vi "test3-FirstChainNodeProcessesAllowedMessages.vi"(8 "error in (no error)":errorcluster, 11 "TestCase in":refnum<class "testcase-CSMChainMode.lvclass">) -> (0 "error out":errorcluster, 3 "TestCase out":refnum<class "testcase-CSMChainMode.lvclass">)   [LabVIEW 2017, in "testcase-CSMChainMode.lvclass"]
uses:
  testcase-CSMChainMode.lvclass
  <vilib>/addons/_JKI Toolkits/VI Tester/TestCase.llb/TestCase.lvclass
  src/user.lib/_NEVSTOP/Communicable State Machine(CSM)/Communicable State Machine.lvlib
  C:/Program Files (x86)/National Instruments/LabVIEW 2017/vi.lib/addons/_JKI Toolkits/VI Tester/TestCase.llb/TestCase.lvclass
panel:
  out "LoopCount":i32
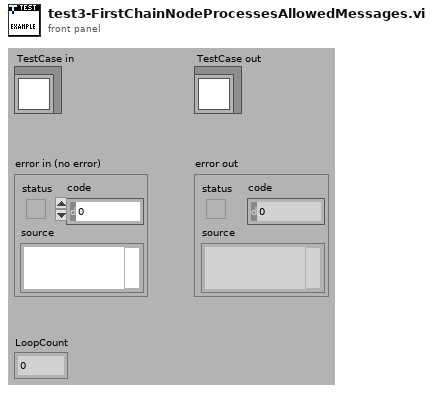
[diagram p1: front panel]
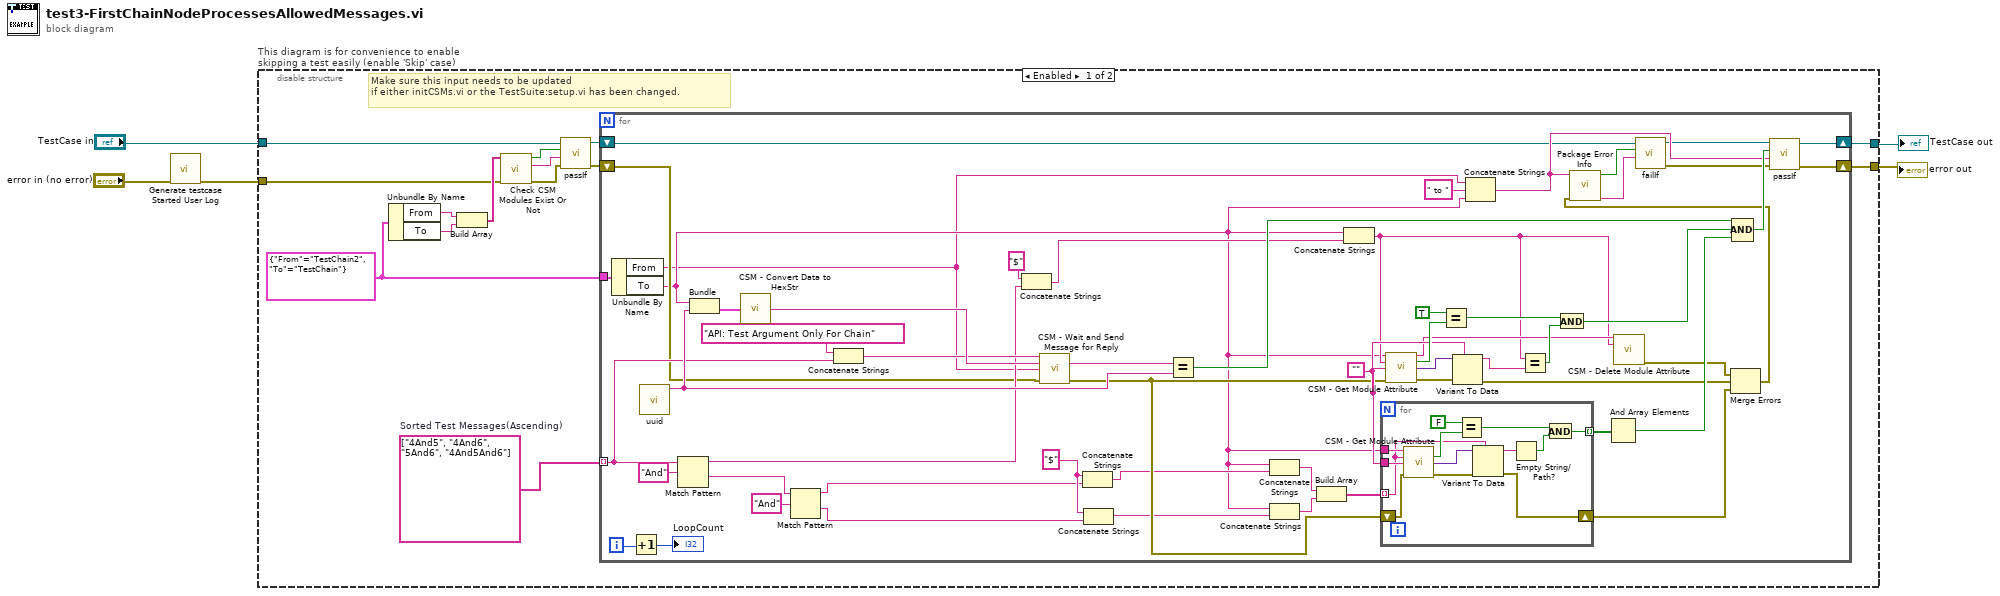
[diagram p0: block diagram]
diagram:
  n1 = call "Generate testcase Started User Log.vi"("Error In"="error in (no error)") -> ("error out"=w1:errorcluster)  [unwired: 10 in]
  n2 = disable-structure "This diagram is for convenience to enable skipping a test easily (enable 'Skip' case)" shown="Enabled" {
    disable-tunnel: "TestCase in" -> [w8 w92]
    disable-tunnel: [w19 w90] -> w2
    disable-tunnel: [w18 w91] -> w4
    disable-tunnel: w1 -> [w7 w89]
    frame Enabled {
      w10 = cluster{"From":string, "To":string} {"From"="TestChain2", "To"="TestChain"} ("Cluster")
      w17 = string[] ["4And5", "4And6", "5And6", "4And5And6"]  # Sorted Test Messages(Ascending)
      # "Make sure this input needs to be updated \nif either initCSMs.vi or the TestSuite:setup.vi has been changed."
      n3 = Unbundle By Name(w10) -> ("From"=w12:string, "To"=w13:string)
      n4 = Build Array(w12, w13) -> (w11:string[])
      n5 = call "Check CSM Modules Exist Or Not.vi"("error in"=w7, "CSM names in"=w11) -> ("error out"=w14:errorcluster, "Debug string"=w15:string, "All Modules Exist?"=w16:bool)  [unwired: 7 in]
      n6 = call-dynamic "passIf.vi"("error in (no error)"=w14, "message (\"\")"=w15, "pass"=w16, "TestCase in"=w8) -> ("error out"=w6:errorcluster, "TestCase out"=w9:refnum<class "testcase-CSMChainMode.lvclass">)  [unwired: 6 in]
      n7 = for {
        tunnel: w10 -> [w75]
        shift-right: [w70] -> w19
        shift-left: w9 -> [w26]
        shift-right: [w69] -> w18
        shift-left: w6 -> [w23]
        tunnel: w17 -> [w37] mode=indexing
        i -> [w49]
        w43 = "$" ("string")
        w58 = ""
        n8 = Unbundle By Name(w75) -> ("From"=w20:string, "To"=w21:string)
        n9 = Increment(x=w49) -> (x+1=→"LoopCount":i32)
        n10 = call "uuid.vi"() -> ("UUID"=w61:string)  [unwired: 11 in]
        n11 = Match Pattern(string=w37, regular expression="And") -> (before substring=w35:string, after substring=w33:string)  [unwired: 1 in, 2 out]
        n12 = Bundle("To"=w21, "UUID"=w61) -> (w74:cluster{"To":string, "UUID":string})  [unwired: 1 in]
        n13 = call "CSM - Convert Data to HexStr.vi"("Variant"=w74) -> ("HEX String (0-9,A-F)"=w73:string)  [unwired: 8 in]
        n14 = Match Pattern(string=w33, regular expression="And") -> (before substring=w32:string, after substring=w31:string)  [unwired: 1 in, 2 out]
        n15 = Concatenate Strings("API: Test Argument Only For Chain" ("State"), w37) -> (w46:string)
        n16 = Concatenate Strings("$" ("string"), w35) -> (w44:string)
        n17 = call "CSM - Wait and Send Message for Reply.vi"("State"=w46, "Arguments (\"\")"=w73, "Target Module"=w20, "Error In (No Error)"=w23) -> ("Response"=w62:string, "error out"=w52:errorcluster)  [unwired: 8 in, 2 out]
        n18 = Concatenate Strings(w43, w32) -> (w42:string)
        n19 = Concatenate Strings(w43, w31) -> (w41:string)
        n20 = Equal?(x=w62, y=w61) -> (x = y?=w72:bool)
        n21 = Concatenate Strings(w21, w42) -> (w57:string)
        n22 = Concatenate Strings(w21, w41) -> (w56:string)
        n23 = Build Array(w57, w56) -> (w55:string[])
        n24 = Concatenate Strings(w21, w44) -> (w39:string)
        n25 = for {
          tunnel: w58 -> [w88]
          tunnel: w21 -> [w83]
          tunnel: w55 -> [w82] mode=indexing
          tunnel: [w78] -> w54 mode=indexing
          shift-right: [w76] -> w50
          shift-left: w52 -> [w77]
          n26 = call "CSM - Get Module Attribute.vi"("CSM Name"=w83, "Attribute"=w82, "Default Value (Empty Variant)"=w88, "Error In"=w77) -> ("Found"=w85:bool, "Value"=w86:variant, "error out"=w87:errorcluster)  [unwired: 7 in, 2 out]
          n27 = Equal?(x=FALSE, y=w85) -> (x = y?=w79:bool)
          n28 = Variant To Data(error in=w87, type=w82, Variant=w86) -> (data=w81:string, error out=w76:errorcluster)
          n29 = Empty String/Path?(string/path=w81) -> (empty?=w80:bool)
          n30 = And(x=w79, y=w80) -> (x .and. y?=w78:bool)
        }
        n31 = call "CSM - Get Module Attribute.vi"("CSM Name"=w21, "Attribute"=w39, "Default Value (Empty Variant)"=w58, "Error In"=w52) -> ("CSM Name (Dup)"=w40:string, "Found"=w68:bool, "Value"=w65:variant, "error out"=w66:errorcluster)  [unwired: 7 in, 1 out]
        n32 = Equal?(x=TRUE, y=w68) -> (x = y?=w64:bool)
        n33 = Variant To Data(error in=w66, type=w58, Variant=w65) -> (data=w60:string, error out=w51:errorcluster)
        n34 = Concatenate Strings(w20, " to " ("string"), w21) -> (w27:string)
        n35 = Equal?(x=w39, y=w60) -> (x = y?=w63:bool)
        n36 = And(x=w64, y=w63) -> (x .and. y?=w59:bool)
        n37 = And Array Elements(Boolean array=w54) -> (logical AND=w53:bool)
        n38 = call "CSM - Delete Module Attribute.vi"("CSM Name"=w40, "Attribute"=w39) -> ("error out"=w38:errorcluster)  [unwired: 10 in, 3 out]
        n39 = Merge Errors(w38, w51, w50) -> (w22:errorcluster)
        n40 = call "Package Error Info.vi"("error in"=w22, "String in"=w27) -> ("packed error info out"=w29:string, "error status"=w30:bool)  [unwired: 8 in]
        n41 = call-dynamic "failIf.vi"("message (\"\")"=w29, "fail"=w30, "TestCase in"=w26) -> ("error out"=w24:errorcluster, "TestCase out"=w25:refnum<class "testcase-CSMChainMode.lvclass">)  [unwired: 7 in]
        n42 = Compound Arithmetic op=AND(w72, w59, w53) -> (w71:bool)
        n43 = call-dynamic "passIf.vi"("error in (no error)"=w24, "message (\"\")"=w27, "pass"=w71, "TestCase in"=w25) -> ("error out"=w69:errorcluster, "TestCase out"=w70:refnum<class "testcase-CSMChainMode.lvclass">)  [unwired: 6 in]
      }
    }
    frame Disabled {
      # "skip test result while test is under development"
      n44 = call <vilib>:"skip.vi"("error in (no error)"=w89, "TestCase in"=w92) -> ("error out"=w91:errorcluster, "TestCase out"=w90:refnum<class "testcase-CSMChainMode.lvclass">)  [unwired: 8 in]
    }
  }
  "error out" <- w4
  "TestCase out" <- w2
